vi "W21_RunPy.vi"() -> ()   [LabVIEW 2018]
doc: "Use this template to build a VI to use as a subVI."
panel:
  out "analysis OK":bool
  out "error out":errorcluster
  out "p":dbl
  out "last line":string
  out "return code":i32
  out "stderr (log)":string
  out "stdout":string
  in  "out":string
  in  "end":string
  in  "start":string
  in  "station":string
  in  "db":string
  in  "yield_report.py":string
  in  "python.exe":string
  # "Set python.exe, yield_report.py, db, station, start, end, out. Paths may contain spaces (quoted in the format string)."
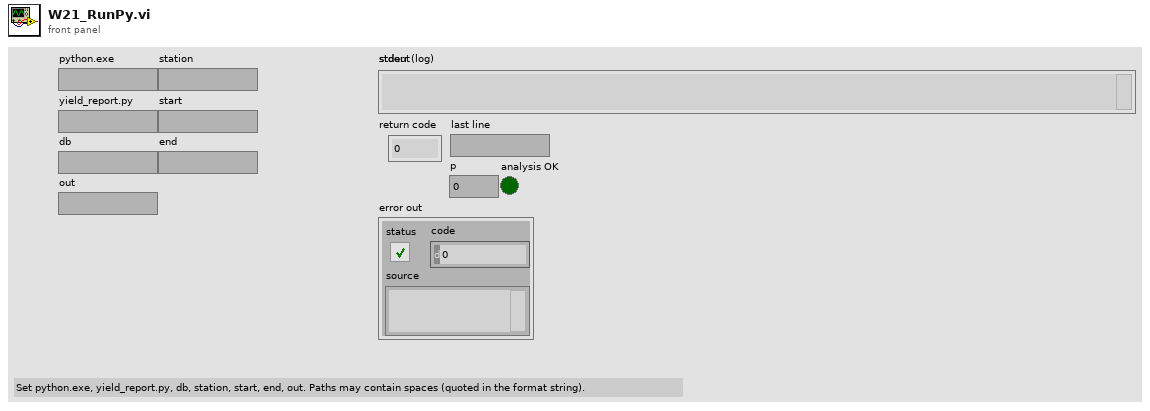
[diagram p1: front panel]
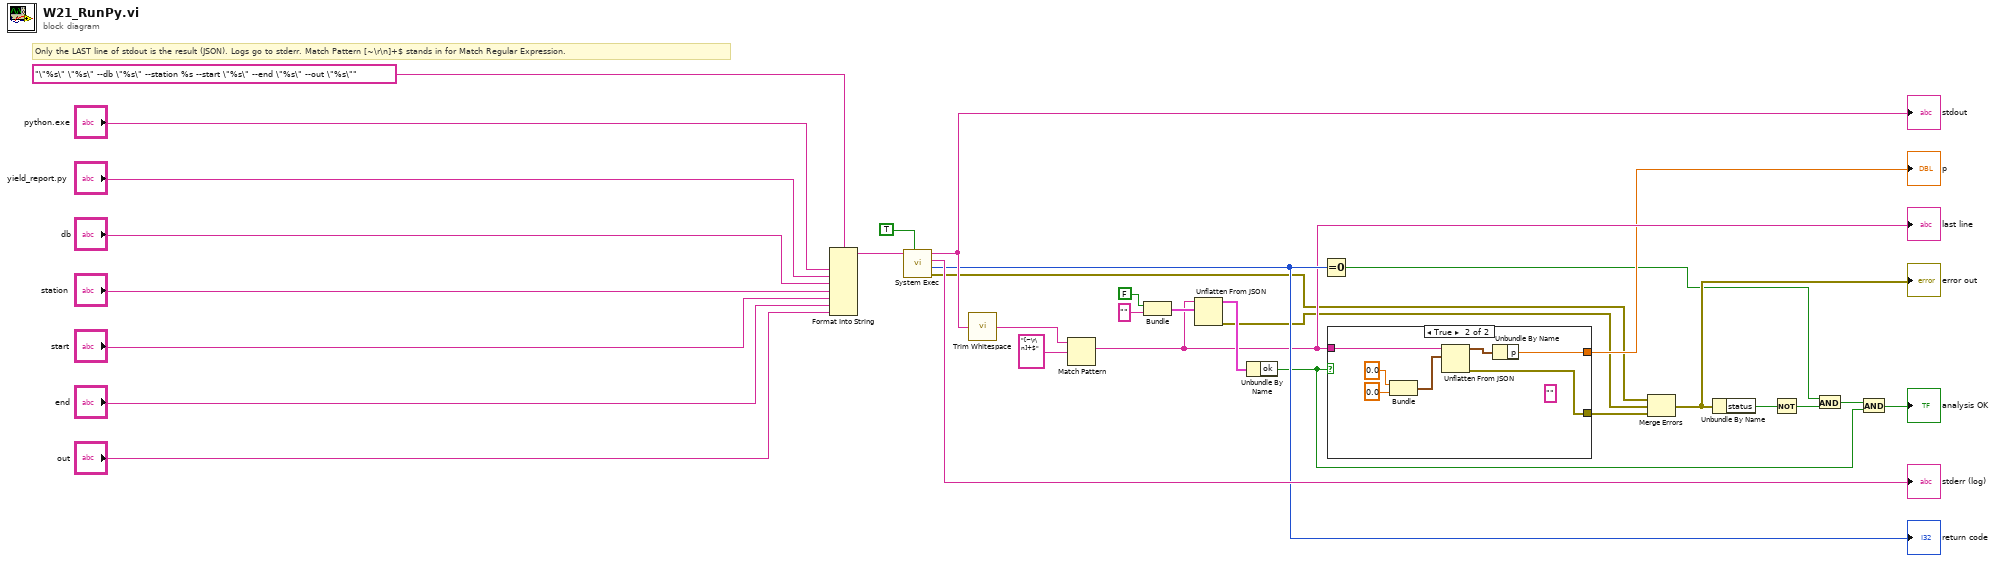
[diagram p0: block diagram]
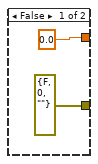
[diagram p2: hidden frame]
diagram:
  # "Only the LAST line of stdout is the result (JSON). Logs go to stderr. Match Pattern [~\\r\\n]+$ stands in for Match Regular Expression."
  n1 = Format Into String(format string="\"%s\" \"%s\" --db \"%s\" --station %s --start \"%s\" --end \"%s\" --out \"%s\"", "python.exe", "yield_report.py", "db", "station", "start", "end", "out") -> (resulting string=w23:string)  [unwired: 2 in, 1 out]
  n2 = call <vilib>:"System Exec.vi"("wait until completion? (T)"=TRUE, "command line"=w23) -> ("error out"=w9:errorcluster, "return code"=w19:i32, "standard error"=→"stderr (log)":string, "standard output"=w21:string)  [unwired: 6 in]
  "stdout" <- w21
  "return code" <- w19
  n3 = call-poly <vilib>:"Trim Whitespace.vi"("string"=w21) -> ("trimmed string"=w18:string)  [unwired: 1 in]
  n4 = Match Pattern(string=w18, regular expression="[~\r\n]+$") -> (match substring=w11:string)  [unwired: 1 in, 3 out]
  "last line" <- w11
  n5 = Bundle("ok"=FALSE, "ver"="") -> (w14:cluster{"ok":bool, "ver":string})  [unwired: 1 in]
  n6 = Unflatten From JSON(JSON string=w11, type and defaults=w14) -> (value=w13:cluster{"ok":bool, "ver":string}, error out=w8:errorcluster)  [unwired: 5 in]
  n7 = Unbundle By Name(w13) -> ("ok"=w12:bool)
  n8 = Equal To 0?(x=w19) -> (x = 0?=w4:bool)
  n9 = case shown="True" w12 {
    tunnel: w11 -> [_ w38]
    tunnel: [0.0 ("x") w35] -> w10
    tunnel: [errorcluster {"status"=FALSE, "code"=0, "source"=""} ("error in (no error)") w34] -> w7
    frame False {
    }
    frame True {
      (unwired) "" ("png")
      n10 = Bundle("p"=0.0, "n"=0.0) -> (w37:cluster{"p":dbl, "n":dbl})  [unwired: 1 in]
      n11 = Unflatten From JSON(JSON string=w38, type and defaults=w37) -> (value=w36:cluster{"p":dbl, "n":dbl}, error out=w34:errorcluster)  [unwired: 5 in]
      n12 = Unbundle By Name(w36) -> ("p"=w35:dbl)
    }
  }
  "p" <- w10
  n13 = Merge Errors(w9, w8, w7) -> (w6:errorcluster)
  "error out" <- w6
  n14 = Unbundle By Name(w6) -> ("status"=w5:bool)
  n15 = Not(x=w5) -> (.not. x?=w3:bool)
  n16 = And(x=w4, y=w3) -> (x .and. y?=w2:bool)
  n17 = And(x=w2, y=w12) -> (x .and. y?=→"analysis OK":bool)
